vi "RemoteVI Capture And Send.vi"(0 "clients":T2(array[cluster]), 5 "hWnd":u64, 7 "cache":T1, 9 "period":dbl=50.0) -> (4 "clients out":T2(array[cluster]), 6 "cache out":T1, 8 "captured?":bool)   [LabVIEW 2020, in "RemoteVI.lvlib"]
doc: "The frame part of one server loop iteration: when at least one client is connected and period ms have passed since the last frame (cache.time), a frame is made once (RemoteVI Capture Frame.vi - the whole window below its title bar, drawn by PrintWindow, no VI Server call, so also while a popup is open) and RemoteVI Send Frame.vi runs for each client (each client's own flow control decides whether it is sent). cache out holds the capture, its size and the tick count of this frame. captured? is TRUE when a frame was made."
uses:
  RemoteVI.lvlib
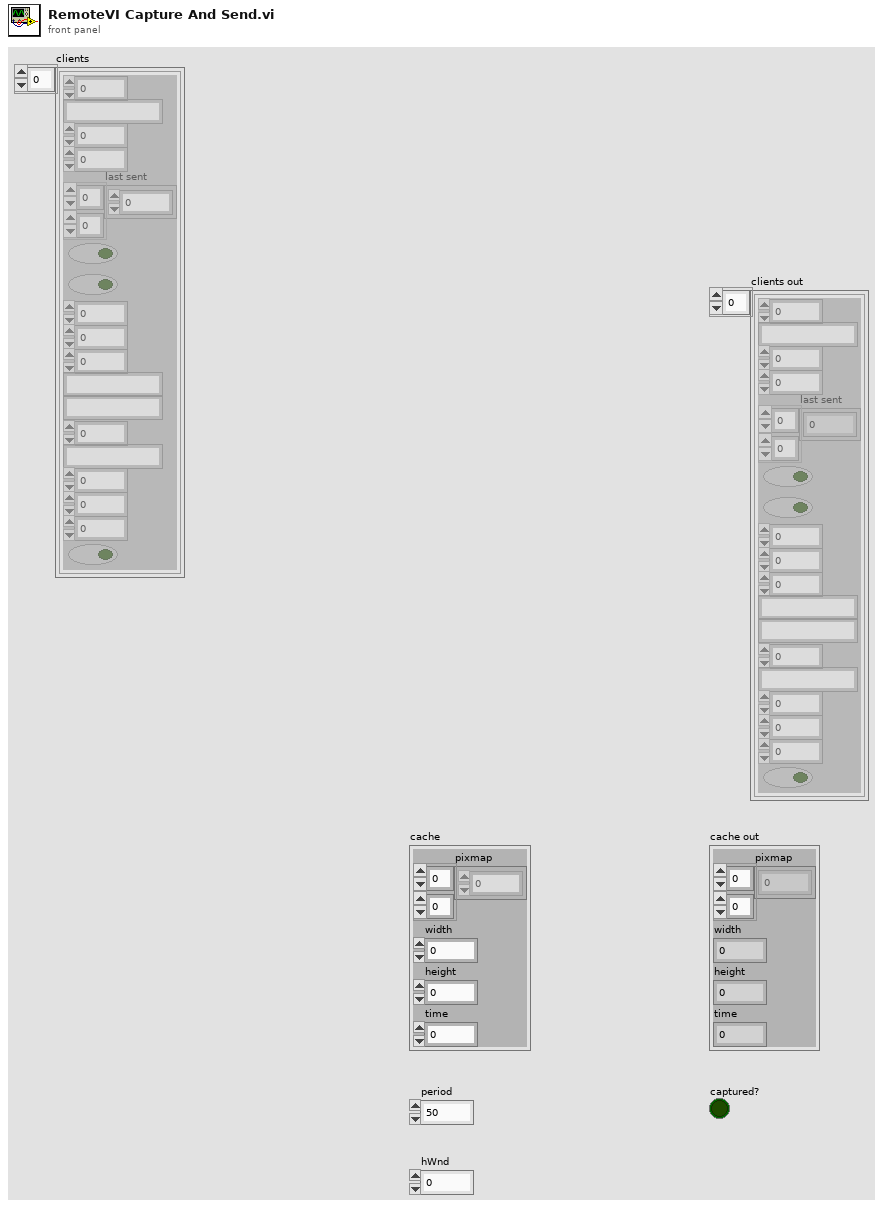
[diagram p1: front panel]
types:
  T1 = cluster{"pixmap":u32[][], "width":i32, "height":i32, "time":u32}
  T2 = cluster{"connection":u32, "rx buffer":string, "seq":u32, "acked":u32, "last sent":u32[][], "tracking":bool, "closed":bool, "mods":u8, "mods set":u8, "popup since":u32, "windows sent":string, "window frames":cluster{"id":u64, "pixels":u32[][]}[], "key window":u64, "address":string, "since":dbl, "last input":dbl, "bytes":dbl, "view only":bool}[]
  T3 = cluster{"connection":u32, "rx buffer":string, "seq":u32, "acked":u32, "last sent":u32[][], "tracking":bool, "closed":bool, "mods":u8, "mods set":u8, "popup since":u32, "windows sent":string, "window frames":cluster{"id":u64, "pixels":u32[][]}[], "key window":u64, "address":string, "since":dbl, "last input":dbl, "bytes":dbl, "view only":bool}
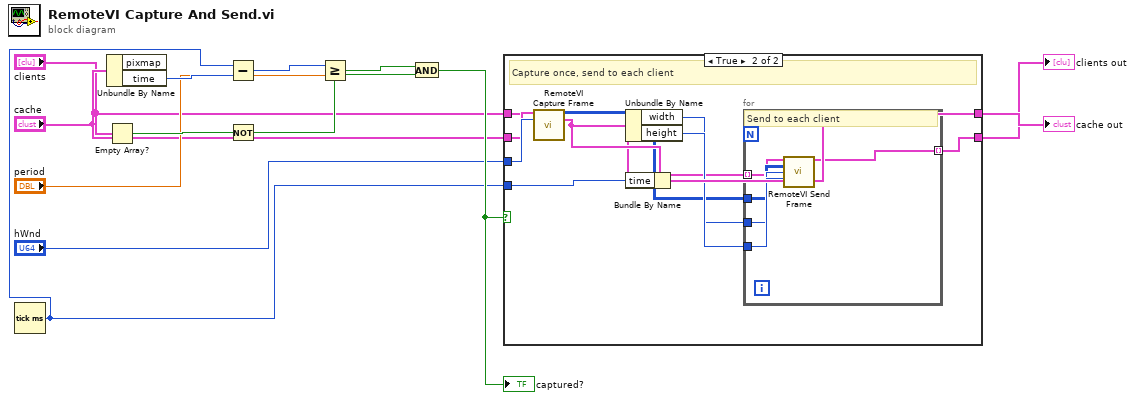
[diagram p0: block diagram]
diagram:
  n1 = Tick Count (ms)() -> (millisecond timer value=w5:u32)
  n2 = Unbundle By Name("cache") -> ("time"=w6:u32)  [unwired: 1 out]
  n3 = Empty Array?(array="clients") -> (empty?=w9:bool)
  n4 = Subtract(x=w5, y=w6) -> (x-y=w7:u32)
  n5 = Not(x=w9) -> (.not. x?=w10:bool)
  n6 = Greater Or Equal?(x=w7, y="period") -> (x >= y?=w8:bool)
  n7 = And(x=w8, y=w10) -> (x .and. y?=w11:bool)
  "captured?" <- w11
  n8 = case shown="True" w11 {
    tunnel: "clients" -> [w14 w16]
    tunnel: "cache" -> [w15 w17]
    tunnel: "hWnd" -> [_ w18]
    tunnel: w5 -> [_ w19]
    tunnel: [w15 w25] -> w13
    tunnel: [w14 w24] -> w12
    frame False {
    }
    frame True {
      # "Capture once, send to each client"
      n9 = call "RemoteVI Capture Frame.vi"("cache"=w17, "hWnd"=w18) -> ("frame"=w20:u32[][], "cache out"=w21:T1)  [unwired: 12 in]
      n10 = Unbundle By Name(w21) -> ("width"=w22:i32, "height"=w23:i32)
      n11 = Bundle By Name(cluster=w21, "time"=w19) -> (w25:T1)
      n12 = for {
        tunnel: w16 -> [w26] mode=indexing
        tunnel: w20 -> [w27]
        tunnel: w22 -> [w28]
        tunnel: w23 -> [w29]
        tunnel: [w30] -> w24 mode=indexing
        # "Send to each client"
        n13 = call "RemoteVI Send Frame.vi"("Client"=w26, "pixmap"=w27, "width"=w28, "height"=w29) -> ("Client out"=w30:T3)  [unwired: 9 in, 2 out]
      }
    }
  }
  "clients out" <- w12
  "cache out" <- w13
